vi "Configure Module.vi"(8 "error in (no error)":errorcluster, 10 "IOV ref in":variant, 11 "9478 in":refnum<class "9478.lvclass">) -> (0 "error out":errorcluster, 2 "IOV ref out":variant, 3 "9478 out":refnum<class "9478.lvclass">)   [LabVIEW 2020, in "Modules.lvlib" / "9478.lvclass"]
uses:
  9478.lvclass
  <resource>/objmgr/cRIO.rc
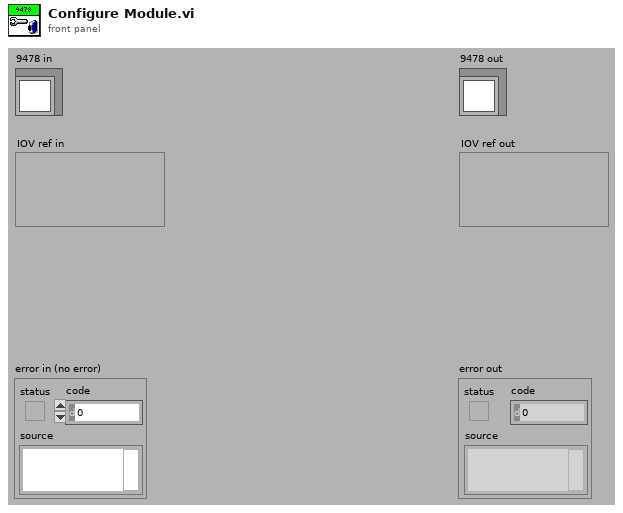
[diagram p1: front panel]
types:
  T1 = typedef "Modules.lvlib/9478.lvclass/Active Limit.ctl" = u8
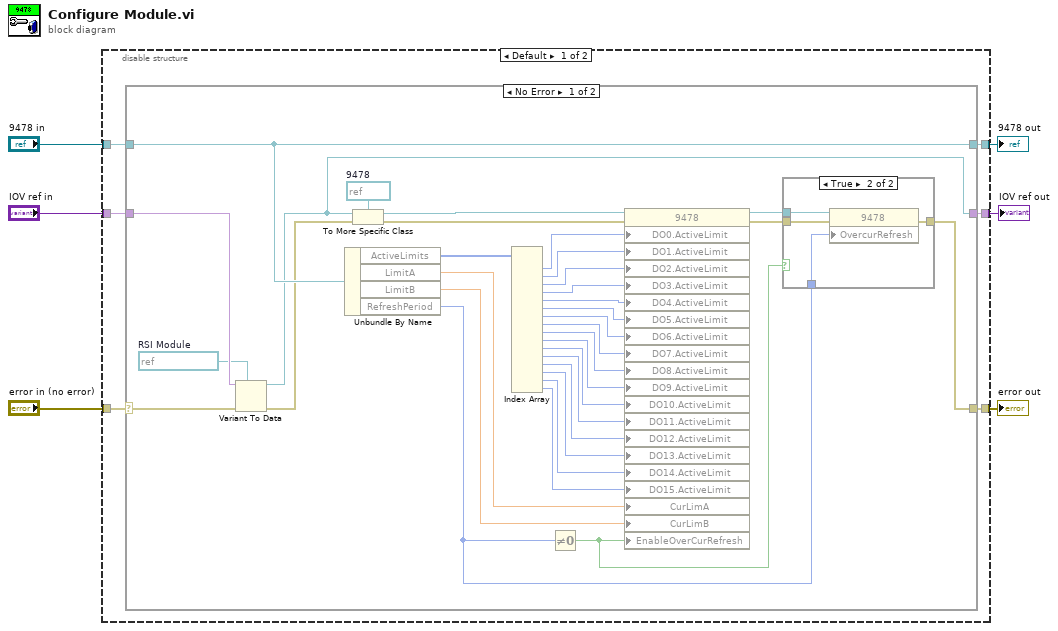
[diagram p0: block diagram]
diagram:
  n1 = disable-structure shown="Default" {
    disable-tunnel: "error in (no error)" -> [w12 w56]
    disable-tunnel: [w11 w56] -> w5
    disable-tunnel: "9478 in" -> [w10 w54]
    disable-tunnel: [w9 w54] -> w3
    disable-tunnel: "IOV ref in" -> [w8 w55]
    disable-tunnel: [w7 w55] -> w1
    frame condition #0 {
      n2 = case shown="No Error" w12 {
        selector: w12 -> [w44 w53]
        tunnel: [w19 w53] -> w11
        tunnel: [w45 w52] -> w9
        tunnel: w10 -> [w45 w52]
        tunnel: w8 -> [w15 w51]
        tunnel: [w14 w51] -> w7
        frame No Error {
          w13 = refnum<k21> refnum  # RSI Module
          w43 = refnum<k21> refnum  # 9478
          n3 = Variant To Data(error in=w44, type=w13, Variant=w15) -> (data=w14:refnum<k21>, error out=w16:errorcluster)
          n4 = Unbundle By Name(w45) -> ("ActiveLimits"=w40:T1[], "LimitA"=w23:dbl, "LimitB"=w22:dbl, "RefreshPeriod"=w17:u8)
          n5 = To More Specific Class(target class=w43, reference=w14, error in=w16) -> (specific class reference=w42:refnum<k21>, error out=w41:errorcluster)
          n6 = Index Array(array=w40) -> (element #1=w39:T1, element #2=w38:T1, element #3=w37:T1, element #4=w36:T1, element #5=w35:T1, element #6=w34:T1, element #7=w33:T1, element #8=w32:T1, element #9=w31:T1, element #10=w30:T1, element #11=w29:T1, element #12=w28:T1, element #13=w27:T1, element #14=w26:T1, element #15=w25:T1, element #16=w24:T1)  [unwired: 16 in]
          n7 = Not Equal To 0?(x=w17) -> (x != 0?=w18:bool)
          n8 = property class="9478"(reference=w42, error in=w41, "DO0.ActiveLimit"=w39, "DO1.ActiveLimit"=w38, "DO2.ActiveLimit"=w37, "DO3.ActiveLimit"=w36, "DO4.ActiveLimit"=w35, "DO5.ActiveLimit"=w34, "DO6.ActiveLimit"=w33, "DO7.ActiveLimit"=w32, "DO8.ActiveLimit"=w31, "DO9.ActiveLimit"=w30, "DO10.ActiveLimit"=w29, "DO11.ActiveLimit"=w28, "DO12.ActiveLimit"=w27, "DO13.ActiveLimit"=w26, "DO14.ActiveLimit"=w25, "DO15.ActiveLimit"=w24, "CurLimA"=w23, "CurLimB"=w22, "EnableOverCurRefresh"=w18) -> (reference out=w21:refnum<k21>, error out=w20:errorcluster)
          n9 = case shown="True" w18 {
            tunnel: w21 -> [_ w50]
            tunnel: w20 -> [w46 w49]
            tunnel: [w46 w48] -> w19
            tunnel: w17 -> [_ w47]
            frame False {
            }
            frame True {
              n10 = property class="9478"(reference=w50, error in=w49, "OvercurRefresh"=w47) -> (error out=w48:errorcluster)  [unwired: 1 out]
            }
          }
        }
        frame Error {
        }
      }
    }
    frame condition #1 (active) {
    }
  }
  "error out" <- w5
  "9478 out" <- w3
  "IOV ref out" <- w1
